vi "lvmcp_move.vi"() -> ()   [LabVIEW 2026]
panel:
  out "error out":errorcluster
  in  "position":cluster{"x":i32, "y":i32}
  in  "owner":refnum<vi>
  in  "reference":refnum<vi>
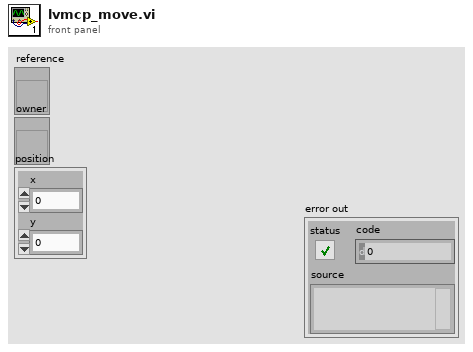
[diagram p1: front panel]
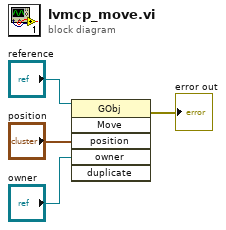
[diagram p0: block diagram]
diagram:
  n1 = invoke class="GObj" method="Move"(reference="reference", "position"="position", "owner"="owner") -> (error out=→"error out":errorcluster)  [unwired: 3 in, 5 out]
